vi "Stop Iterations.vi"(8 "error in (no error)":errorcluster, 11 "Iterator Actor in":refnum<class "Abstract Iterator Actor.lvclass">) -> (0 "error out":errorcluster, 3 "Iterator Actor out":refnum<class "Abstract Iterator Actor.lvclass">)   [LabVIEW 2023, in "Iterator Actor.lvlib" / "Abstract Iterator Actor.lvclass"]
doc: "Stops all the subsequent iterations."
uses:
  Abstract Iterator Actor.lvclass
  C:/Program Files/National Instruments/LabVIEW 2023/vi.lib/ActorFramework/Actor/Actor.lvclass
  Abstract Iterator Actor.lvclass/Abstract Iterator Actor.ctl
  <vilib>/ActorFramework/Actor/Actor.lvclass/Actor.ctl
  <vilib>/ActorFramework/Report Error Msg/Report Error Msg.lvclass/Report Error Msg.ctl
  <vilib>/ActorFramework/Message Enqueuer/Message Enqueuer.lvclass/Message Enqueuer.ctl
  <vilib>/ActorFramework/Message Enqueuer/Enqueue.vi
  <vilib>/ActorFramework/Report Error Msg/Report Error Msg.lvclass
  C:/Program Files/National Instruments/LabVIEW 2023/vi.lib/ActorFramework/Message/Message.lvclass
  <vilib>/Utility/error.llb/Error Cluster From Error Code.vi
  <vilib>/ActorFramework/Message Priority Queue/Priority Enqueue.vi
  <vilib>/ErrorRing/Error Ring.xnode
  <vilib>/ActorFramework/Actor/Actor.lvclass
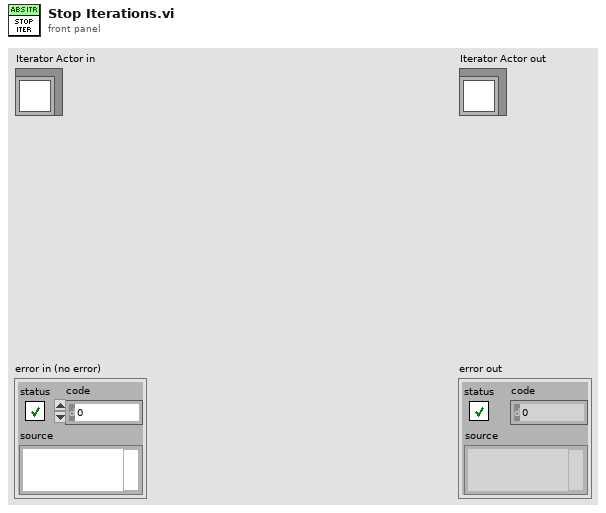
[diagram p1: front panel]
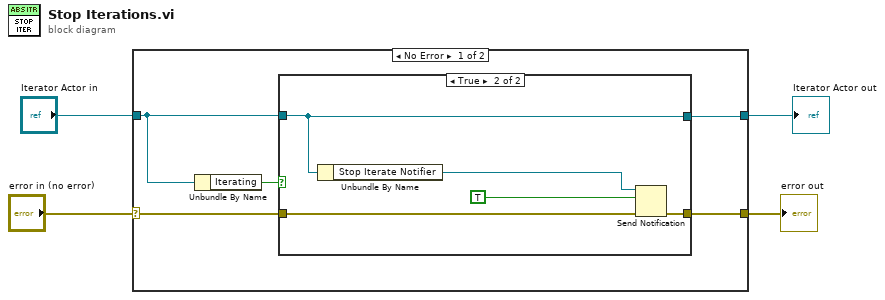
[diagram p0: block diagram]
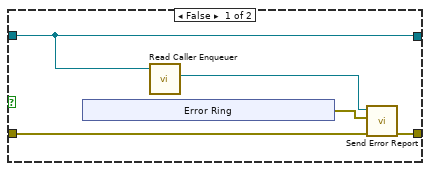
[diagram p2: hidden frame]
diagram:
  n1 = case shown="No Error" "error in (no error)" {
    selector: "error in (no error)" -> [w8 w25]
    tunnel: [w9 w25] -> w3
    tunnel: [w5 w24] -> w1
    tunnel: "Iterator Actor in" -> [w6 w24]
    frame No Error {
      n2 = Unbundle By Name(w6) -> ("Iterating"=w7:bool)
      n3 = case shown="True" w7 {
        tunnel: [w11 w23] -> w9
        tunnel: w8 -> [w12 w22]
        tunnel: w6 -> [w10 w19]
        tunnel: [w10 w19] -> w5
        frame False {
          n4 = xnode "Error Ring"() -> ("error out"=w14:errorcluster)
          n5 = call <vilib>:"Read Caller Enqueuer.vi"("Actor"=w10) -> ("Caller Enqueuer"=w13:refnum<class "Message Enqueuer.lvclass">)  [unwired: 10 in]
          n6 = call <vilib>:"Send Error Report.vi"("error in (no error)"=w12, "Error From Sender"=w14, "Message Enqueuer"=w13) -> ("error out"=w11:errorcluster)  [unwired: 8 in]
        }
        frame True {
          n7 = Unbundle By Name(w19) -> ("Stop Iterate Notifier"=w21:refnum<notifier>)
          n8 = Send Notification(notification=TRUE, notifier=w21, error in (no error)=w22) -> (error out=w23:errorcluster)  [unwired: 1 out]
        }
      }
    }
    frame Error {
    }
  }
  "error out" <- w3
  "Iterator Actor out" <- w1
